vi "Day 21.vi"() -> ()   [LabVIEW 2021]
uses:
  Day 21-Turn Cluster.ctl
  Day 21-Player Turn.ctl
panel:
  out "Dice Roll Count":u64
  out "Player 2 Score":u64
  out "Player 1 Score":u64
  in  "Player 2 Starting Position":u64=3
  in  "Player 1 Starting Position":u64=10
  out "Solution":u64
  # "Example:\nPlayer 1 starting position: 4\nPlayer 2 starting position: 8"
  # "Input:\nPlayer 1 starting position: 10\nPlayer 2 starting position: 3"
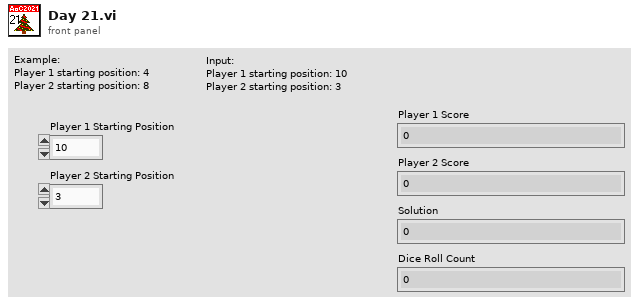
[diagram p1: front panel]
types:
  T1 = typedef "Day 21-Turn Cluster.ctl" = cluster{"Player 1 Position":u64, "Player 1 Score":u64, "Player 2 Position":u64, "Player 2 Score":u64, "Player Turn":T2}
  T2 = typedef "Day 21-Player Turn.ctl" = enum16{"Player 1", "Player 2"}
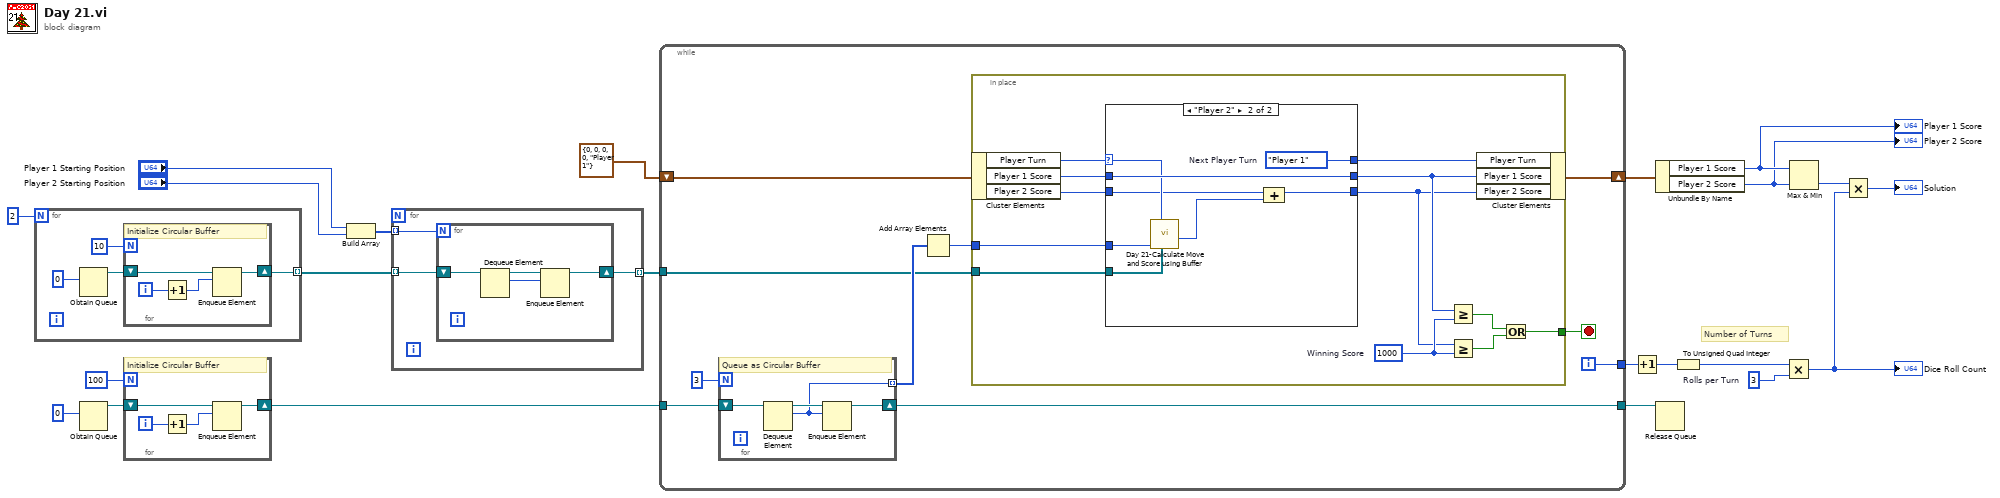
[diagram p0: block diagram]
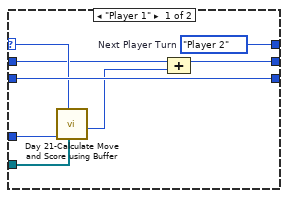
[diagram p2: hidden frame]
diagram:
  w11 = u64 3  # Rolls per Turn
  # "Number of Turns"
  n1 = for {
    N: 2 -> [_]
    tunnel: [w23] -> w4 mode=indexing
    n2 = Obtain Queue(element data type=u64 0) -> (queue out=w25:refnum<queue>)  [unwired: 4 in, 2 out]
    n3 = for {
      N: 10 -> [_]
      shift-right: [w27] -> w23
      shift-left: w25 -> [w30]
      i -> [w29]
      # "Initialize Circular Buffer"
      n4 = Increment(x=w29) -> (x+1=w28:i32)
      n5 = Enqueue Element(queue=w30, element=w28) -> (queue out=w27:refnum<queue>)  [unwired: 2 in, 2 out]
    }
  }
  n6 = Obtain Queue(element data type=u64 0) -> (queue out=w16:refnum<queue>)  [unwired: 4 in, 2 out]
  n7 = for {
    N: 100 -> [_]
    shift-right: [w31] -> w14
    shift-left: w16 -> [w34]
    i -> [w33]
    # "Initialize Circular Buffer"
    n8 = Increment(x=w33) -> (x+1=w32:i32)
    n9 = Enqueue Element(queue=w34, element=w32) -> (queue out=w31:refnum<queue>)  [unwired: 2 in, 2 out]
  }
  n10 = Build Array("Player 1 Starting Position", "Player 2 Starting Position") -> (w3:u64[])
  n11 = for {
    tunnel: w4 -> [w37] mode=indexing
    tunnel: w3 -> [w36] mode=indexing
    tunnel: [w35] -> w2 mode=indexing
    n12 = for {
      N: w36 -> [_]
      shift-right: [w39] -> w35
      shift-left: w37 -> [w41]
      n13 = Dequeue Element(queue=w41) -> (queue out=w40:refnum<queue>, element=w38:u64)  [unwired: 2 in, 2 out]
      n14 = Enqueue Element(queue=w40, element=w38) -> (queue out=w39:refnum<queue>)  [unwired: 2 in, 2 out]
    }
  }
  n15 = while {
    shift-right: [w49] -> w22
    shift-left: T1 {"Player 1 Position"=0, "Player 1 Score"=0, "Player 2 Position"=0, "Player 2 Score"=0, "Player Turn"=enum."Player 1"} ("State") -> [w51]
    tunnel: w14 -> [w46]
    tunnel: [w45] -> w13
    tunnel: [w43] -> w12
    tunnel: w2 -> [w42]
    i -> [w43]
    stop <- w48 stop-if-true
    n16 = for {
      N: 3 -> [_]
      tunnel: [w53] -> w44 mode=indexing
      shift-right: [w52] -> w45
      shift-left: w46 -> [w55]
      # "Queue as Circular Buffer"
      n17 = Dequeue Element(queue=w55) -> (queue out=w54:refnum<queue>, element=w53:u64)  [unwired: 2 in, 2 out]
      n18 = Enqueue Element(queue=w54, element=w53) -> (queue out=w52:refnum<queue>)  [unwired: 2 in, 2 out]
    }
    n19 = Add Array Elements(numeric array=w44) -> (sum=w50:u64)
    n20 = in-place {
      in-place-border: [w63] -> w48
      in-place-border: w50 -> [w57]
      in-place-border: w42 -> [w56]
      w64 = u64 1000  # Winning Score
      n21 = in-place-cluster #1(w51) -> ("Player Turn"=w67:T2, "Player 1 Score"=w66:u64, "Player 2 Score"=w65:u64)
      n22 = case shown="\"Player 2\"" w67 {
        selector: w67 -> [w70 w78]
        tunnel: w57 -> [w73 w81]
        tunnel: w66 -> [w68 w80]
        tunnel: [w69 w80] -> w59
        tunnel: [w75 w77] -> w58
        tunnel: w65 -> [w75 w76]
        tunnel: [w74 w83] -> w62
        tunnel: w56 -> [w71 w79]
        frame "Player 1" {
          w74 = Day_21-Player_Turn."Player 2"  # Next Player Turn
          n23 = call "Day 21-Calculate Move and Score using Buffer.vi"("Game Board Buffer"=w71, "Player Turn"=w70, "Dice Roll Sum"=w73) -> ("Points Earned"=w72:u64)  [unwired: 8 in]
          n24 = Compound Arithmetic op=ADD(w68, w72) -> (w69:u64)
        }
        frame "Player 2" {
          w83 = Day_21-Player_Turn."Player 1"  # Next Player Turn
          n25 = call "Day 21-Calculate Move and Score using Buffer.vi"("Game Board Buffer"=w79, "Player Turn"=w78, "Dice Roll Sum"=w81) -> ("Points Earned"=w82:u64)  [unwired: 8 in]
          n26 = Compound Arithmetic op=ADD(w76, w82) -> (w77:u64)
        }
      }
      n27 = Greater Or Equal?(x=w59, y=w64) -> (x >= y?=w61:bool)
      n28 = Greater Or Equal?(x=w58, y=w64) -> (x >= y?=w60:bool)
      n29 = in-place-cluster #1("Player Turn"=w62, "Player 1 Score"=w59, "Player 2 Score"=w58) -> (w49:T1)
      n30 = Or(x=w61, y=w60) -> (x .or. y?=w63:bool)
    }
  }
  n31 = Increment(x=w12) -> (x+1=w8:i32)
  n32 = Unbundle By Name(w22) -> ("Player 1 Score"=w21:u64, "Player 2 Score"=w20:u64)
  "Player 1 Score" <- w21
  "Player 2 Score" <- w20
  n33 = Release Queue(queue=w13) -> ()  [unwired: 2 in, 3 out]
  n34 = To Unsigned Quad Integer(1:w8) -> (0:w9:u64)
  n35 = Multiply(x=w9, y=w11) -> (x*y=w10:u64)
  "Dice Roll Count" <- w10
  n36 = Max & Min(x=w21, y=w20) -> (min(x,y)=w19:u64)  [unwired: 1 out]
  n37 = Multiply(x=w19, y=w10) -> (x*y=→"Solution":u64)
